vi "PicoScope2000aGetValuesOverlappedBulk.vi"(5 "Segment Range":T1 {"toSegmentIndex" format="%.4p"; "fromSegmentIndex" format="%.4p"}, 7 "Buffer and Transfer Settings":T2={"startIndex"=0, "Samples"=1000, "Down Sample Ratio"=1, "Down-Sample Mode"=1} {"Down-Sample Mode" items=["None"=2147483648, "Aggregate"=1, "Decimate"=2, "Average"=4]; "Down Sample Ratio" step=1; "Samples" format="%_6p"}, 8 "error in (no error)":errorcluster, 11 "handle in":i16) -> (0 "error out":errorcluster, 3 "handle out":i16, 4 "overflow":i16[](array[numeric]) format="%010b", 6 "noOfSamples":u64)   [LabVIEW 2010]
doc: "Calls GetValuesOverlappedBulk"
uses:
  ps2000a.dll
  shared/Buffer and Transfer Settings.ctl
  shared/Segment Range.ctl
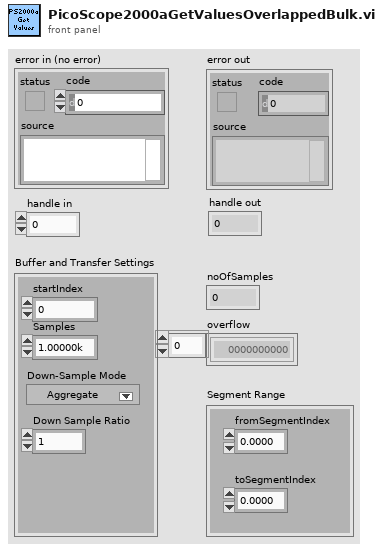
[diagram p1: front panel]
types:
  T1 = typedef "Segment Range.ctl" = cluster{"fromSegmentIndex":u64, "toSegmentIndex":u64}
  T2 = typedef "Buffer and Transfer Settings.ctl" = cluster{"startIndex":u64, "Samples":u64, "Down Sample Ratio":u64, "Down-Sample Mode":u32}
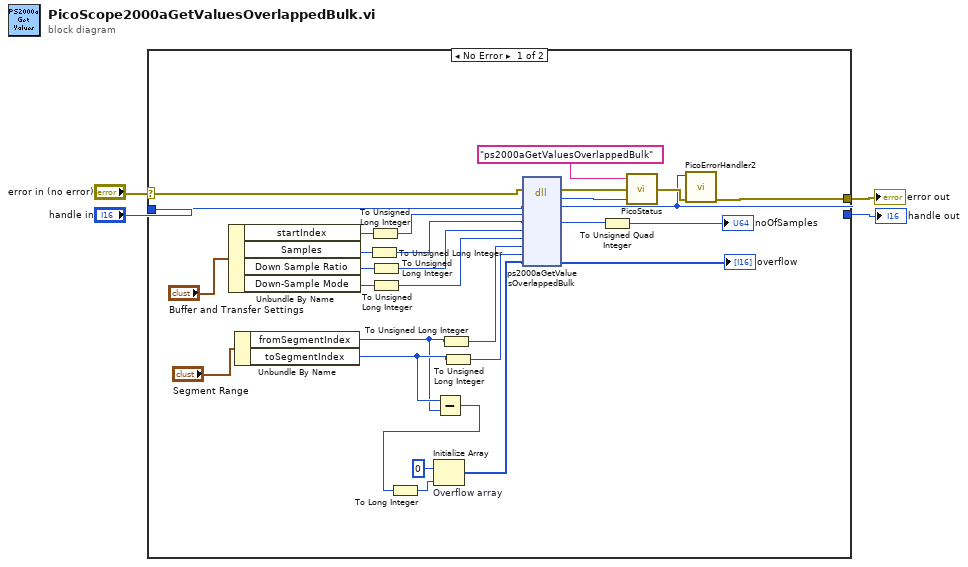
[diagram p0: block diagram]
diagram:
  n1 = case shown="No Error" "error in (no error)" {
    selector: "error in (no error)" -> [w20 w34]
    tunnel: "handle in" -> [w21 w35]
    tunnel: [w27 w35] -> w4
    tunnel: [w30 w34] -> w3
    frame No Error {
      n2 = Unbundle By Name("Buffer and Transfer Settings") -> ("startIndex"=w14:u64, "Samples"=w12:u64, "Down Sample Ratio"=w11:u64, "Down-Sample Mode"=w10:u32)
      n3 = Unbundle By Name("Segment Range") -> ("fromSegmentIndex"=w17:u64, "toSegmentIndex"=w18:u64)
      n4 = To Unsigned Long Integer(number=w12) -> (unsigned 32bit integer=w9:u32)
      n5 = To Unsigned Long Integer(number=w14) -> (unsigned 32bit integer=w13:u32)
      n6 = To Unsigned Long Integer(number=w11) -> (unsigned 32bit integer=w8:u32)
      n7 = To Unsigned Long Integer(number=w10) -> (unsigned 32bit integer=w7:u32)
      n8 = Subtract(x=w18, y=w17) -> (x-y=w22:u64)
      n9 = To Long Integer(number=w22) -> (32bit integer=w24:i32)
      n10 = Initialize Array "Overflow array"(i16 0 ("element"), w24) -> (w23:i16[])
      n11 = To Unsigned Long Integer(number=w17) -> (unsigned 32bit integer=w16:u32)
      n12 = To Unsigned Long Integer(number=w18) -> (unsigned 32bit integer=w15:u32)
      n13 = dll-call lib="ps2000a.dll" fn="ps2000aGetValuesOverlappedBulk" ("ps3000.dll:_ps3000_open_unit@0")(error in=w20, "handle"=w21, "startIndex"=w13, "noOfSamples"=w9, "downSampleRatio"=w8, "downSampleRatioMode"=w7, "fromSegmentIndex"=w16, "toSegmentIndex"=w15, "overflow"=w23) -> (error out=w28:errorcluster, "PICO_STATUS"=w26:u32, "handle"=w27:i16, "noOfSamples"=w5:u32, "overflow"=→"overflow":i16[])  [unwired: 7 in, 1 out]
      n14 = To Unsigned Quad Integer(1:w5) -> (0:→"noOfSamples":u64)
      n15 = call "PicoStatus.vi"("PICO STATUS"=w26, "error in"=w28, "source"="ps2000aGetValuesOverlappedBulk") -> ("error out"=w33:errorcluster)
      n16 = call "PicoErrorHandler2.vi"("error in (no error)"=w33, "handle In"=w27) -> ("error out"=w30:errorcluster)  [unwired: 9 in]
    }
    frame Error {
    }
  }
  "error out" <- w3
  "handle out" <- w4
